vi "VM - Get list of variables.vi"(6 "error in":errorcluster, 7 "reverse? (F)":bool, 8 "sort":enum16{"don't sort", "name", "type"}(ring), 9 "VC Handle":T2=-1) -> (0 "error out":errorcluster, 1 "err code":T1 items=["No error", "Invalid variable type", "Variable not found", "Variable already exists", "Invalid context handle", "Input error", "Invalid data format", "No history attached", "History already attached", "Invalid history parameters", "Wrong variable name", "Wrong alias name", "Non-unique alias", "Alias not found", "No alias associated", "Alias already associated", "Wrong context name", "Non-unique context name", "Context name not found", "Invalid parameter", "Generic error", "Memory Full", "Unrecognized LV error", "Unknown error code"], 2 "list of variables":cluster{"name":string, "type":u32}[](array[cluster]), 3 "dup VC Handle":T2=-1)   [LabVIEW 2021]
doc: "<b>*** DEPRECATED ***</b>\n\nThe VI returns a list of variables in a given context. The list contains both variable names and types. See online help for the VI for more information.\n\n<VC Handle> control should contain a handle of context. If the handle corresponds to an opened context, the VI returns a list of all variables residing in the context. To obtain a list of global variables, <VC Handle> has to contain -1 (by default).\n\n::: CalcExpress Toolkit :::\nCopyright (c) 2000-2026 Konstantin Shifershteyn. All rights reserved."
uses:
  cetypes.llb/VarMan Variable Context Handle.ctl
  cetypes.llb/VarMan Error Code.ctl
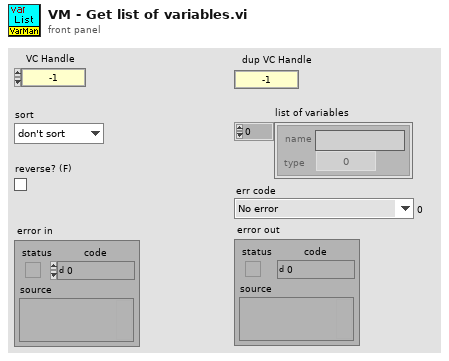
[diagram p1: front panel]
types:
  T1 = typedef "VarMan Error Code.ctl" = u16
  T2 = typedef "VarMan Variable Context Handle.ctl" = i32
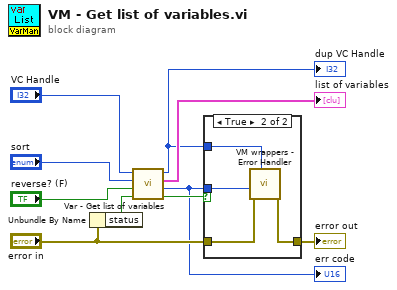
[diagram p0: block diagram]
diagram:
  n1 = Unbundle By Name("error in") -> ("status"=w6:bool)
  n2 = call "Var - Get list of variables"("error in"=w6, "reverse? (F)"="reverse? (F)", "sort"="sort", "VC Handle"="VC Handle") -> ("error out"=w5:bool, "err code"=w2:T1, "list of variables"=→"list of variables":cluster{"name":string, "type":u32}[], "dup VC Handle"=w1:T2)  [unwired: 2 in]
  "dup VC Handle" <- w1
  "err code" <- w2
  n3 = case shown="True" w5 {
    tunnel: [w11 w15] -> w8
    tunnel: "error in" -> [w11 w14]
    tunnel: w2 -> [_ w13]
    tunnel: w1 -> [_ w12]
    frame False {
    }
    frame True {
      n4 = call "VM wrappers - Error Handler.vi"("VC Handle"=w12, "error before"=w14, "VarMan error"=w13) -> ("error out"=w15:errorcluster)  [unwired: 7 in, 1 out]
    }
  }
  "error out" <- w8
